vi "Main.vi"() -> ()   [LabVIEW 2026]
uses:
  <vilib>/Instr/_visa.llb/VISA Configure Serial Port (Instr).vi
panel:
  out "Errores CRC":dbl
  out "Tramas OK":dbl
  out "Estado":string
  out "SALIDA PWM":dbl(graph)
  in  "Modo":bool=TRUE
  in  "RESET":bool
  out "Maquina":T1(ring)
  in  "EMERGENCIA":bool
  in  "PWM":dbl min=0.0 max=100.0
  out "SP Vs ALTURA":cluster{dbl, dbl}(graph)
  out "PING PONG":dbl(slide) scale=0.0..50.0
  out "PID":enum16{"NO CONFIGURADO", "CONFIGURADO"}(ring)
  out "error out":errorcluster
  out "Enum":enum16{"DESCONECTADO", "CONECTADO"}(ring)
  out "ESTADO  SYS":enum16{"DETENIDO", "EJECUTANDO", "ERROR"}(ring)
  in  "PARADA":bool
  in  "INICIO":bool
  out "PID":string
  in  "SP":dbl=25.0 min=0.0 max=100.0
  in  "KD":dbl=0.07 min=0.0 max=65535.0
  in  "KI":dbl=0.14 min=0.0 max=65535.0
  in  "KP":dbl=3.9 min=0.0 max=65535.0
  in  "PID":bool
  out "PWM":dbl format="%.2g"
  out "ERROR":dbl format="%.2g"
  out "ALTURA":dbl format="%.2g"
  out "SP":dbl format="%.2f"
  out "array":string[][](array[string])
  out "Procesar":string
  in  "Stop Simulation":bool
  in  "Numeric":u32=115200
  in  "VISA resource name":refnum<visa-resource-name>="COM12"
  out "Iteracion":i32
  # "Sistema Levitador Neumático"
  # "Planta"
  # "Grafico en Tiempo Real"
  # "COMUNICACIÓN"
  # "ESTADO DEL SISTEMA"
  # "Estado :"
  # "Puerto :"
  # "Comunicación :"
  # "Baud :"
  # "Estado PID :"
  # "CONFIGURACIÓN PID"
  # "VARIABLES EN TIEMPO REAL"
  # "KP :"
  # "KI  :"
  # "KD :"
  # "AUTO"
  # "MANUAL"
  # "SP :"
  # "PWM :"
  # "Mensaje a Procesar :"
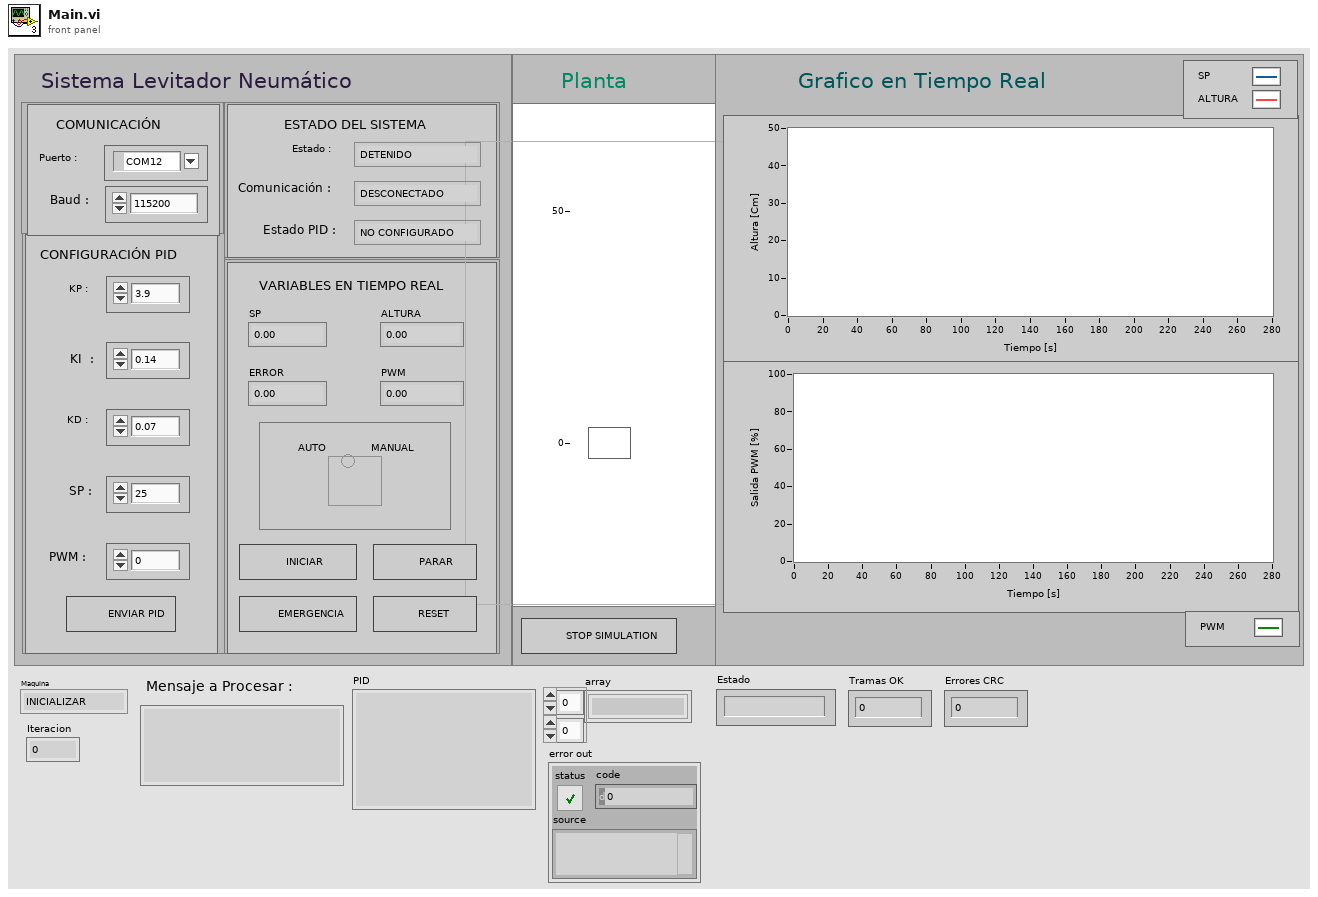
[diagram p1: front panel]
types:
  T1 = enum16{"INICIALIZAR", "ESPERA", "ENVIAR_MODO", "ENVIAR_SP", "ENVIAR_PID", "RECIBIR", "PROCESAR", "ENVIAR_RESET", "ENVIAR_RUN", "ENVIAR_STOP", "ENVIAR_EMERGENCIA_ON", "ENVIAR_EMERGENCIA_OFF", "ERROR", "CERRAR"}
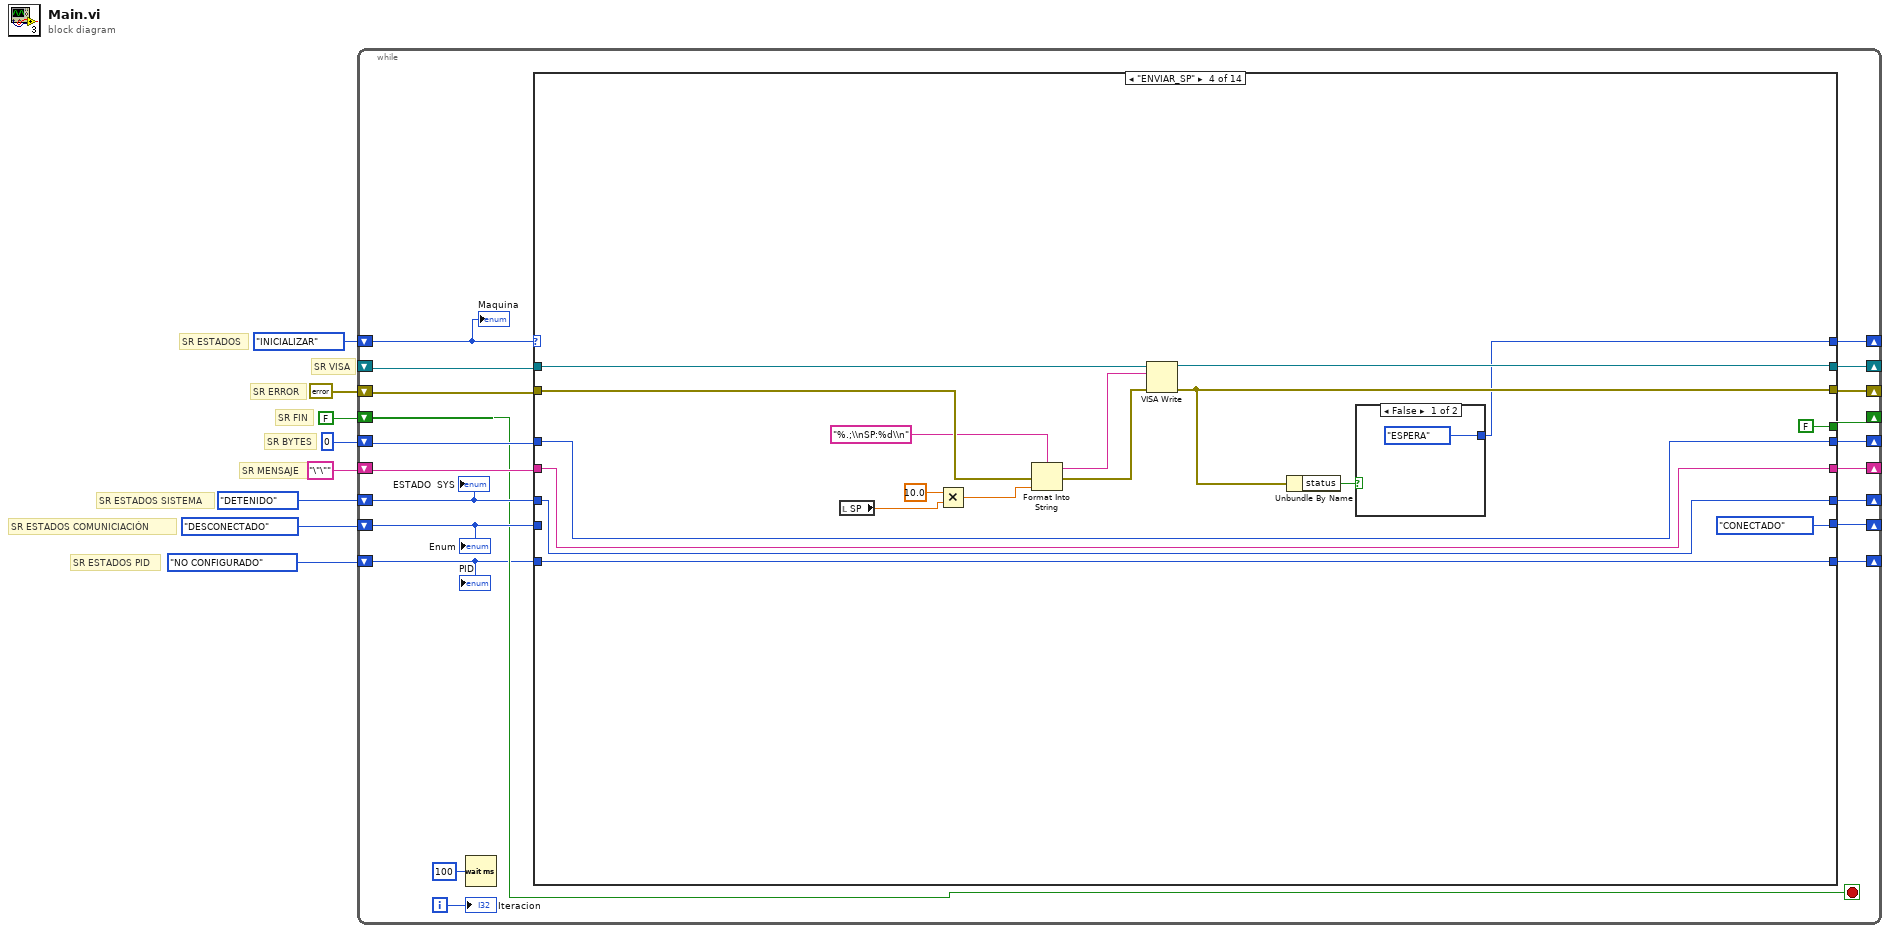
[diagram p0: block diagram]
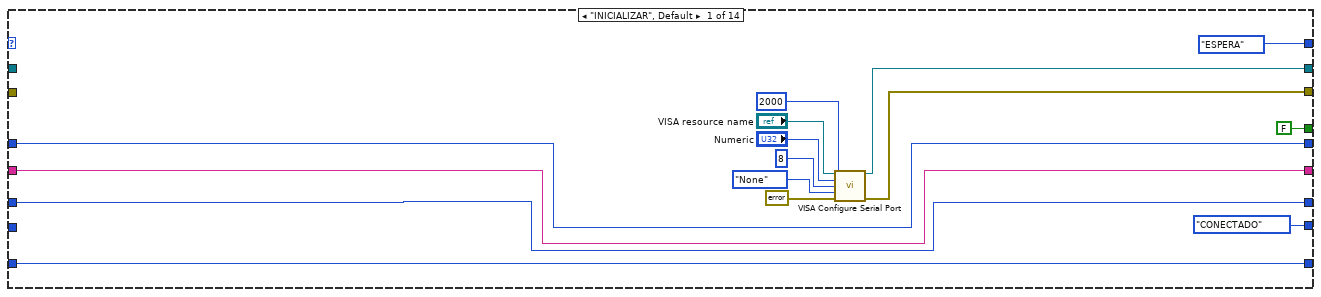
[diagram p2: hidden frame]
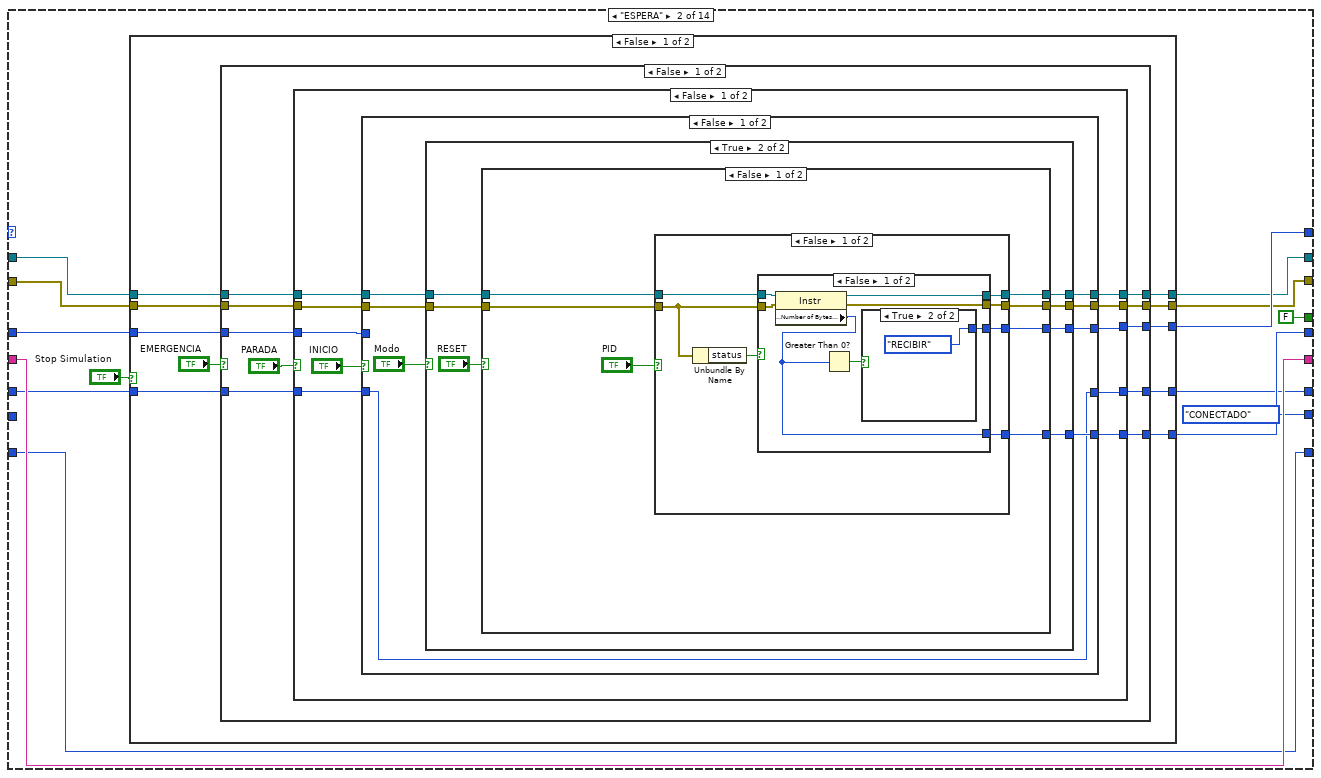
[diagram p3: hidden frame]
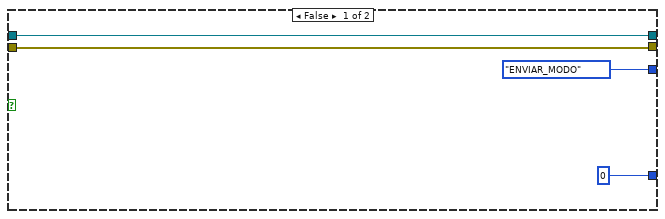
[diagram p4: hidden frame]
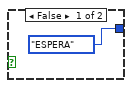
[diagram p5: hidden frame]
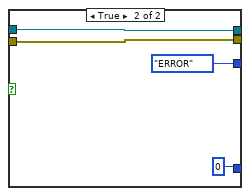
[diagram p6: hidden frame]
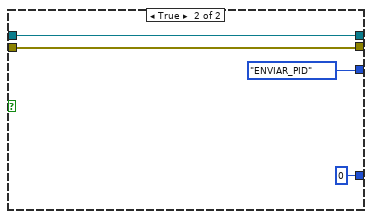
[diagram p7: hidden frame]
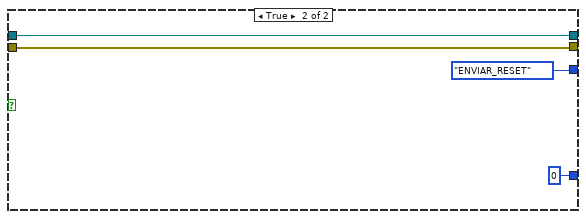
[diagram p8: hidden frame]
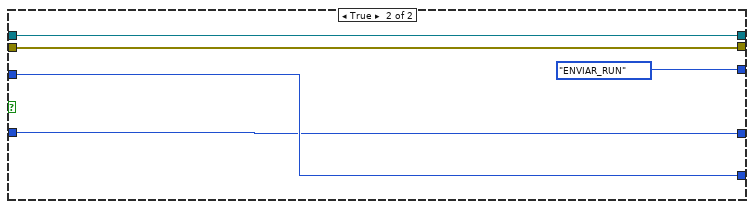
[diagram p9: hidden frame]
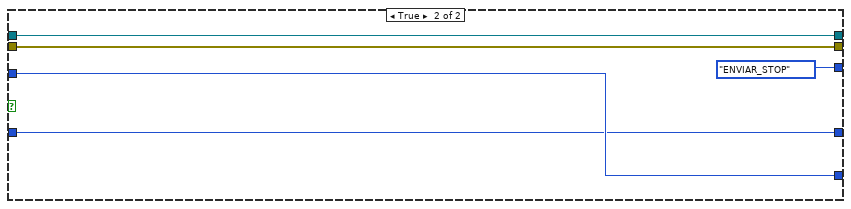
[diagram p10: hidden frame]
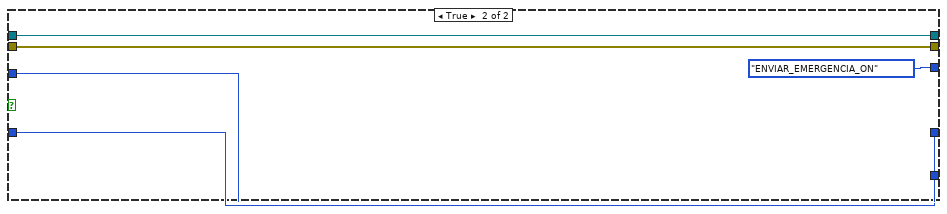
[diagram p11: hidden frame]
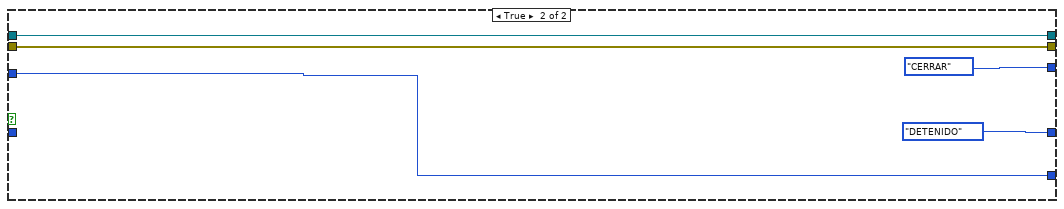
[diagram p12: hidden frame]
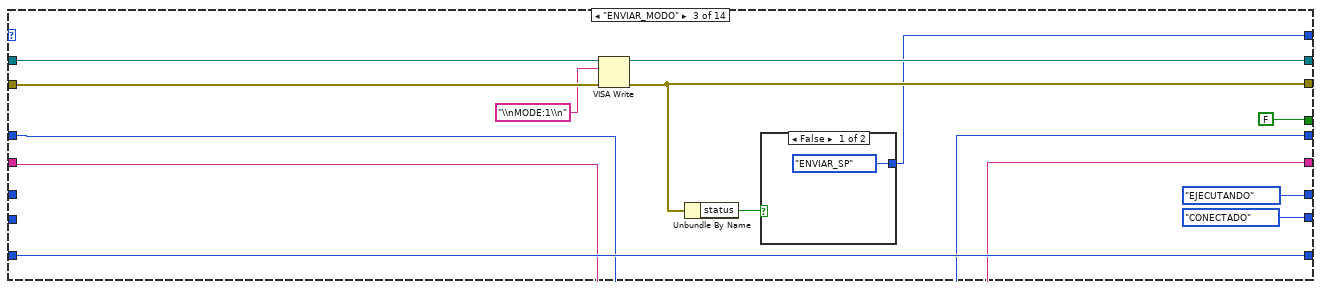
[diagram p13: hidden frame]
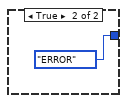
[diagram p14: hidden frame]
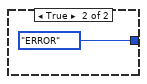
[diagram p15: hidden frame]
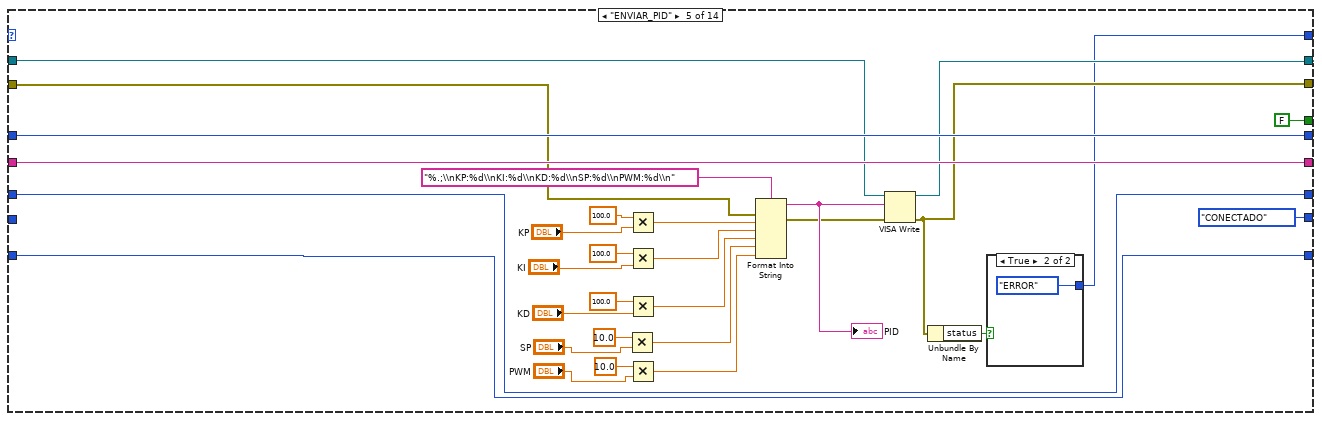
[diagram p16: hidden frame]
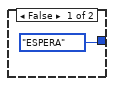
[diagram p17: hidden frame]
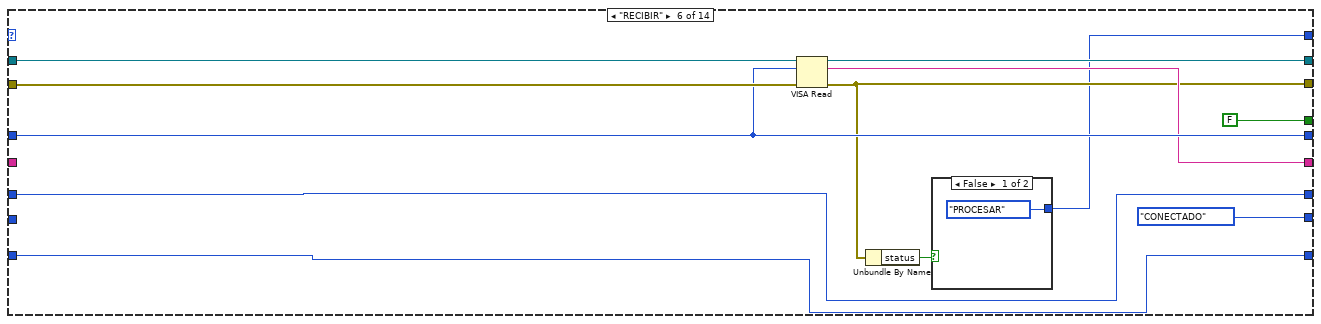
[diagram p18: hidden frame]
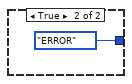
[diagram p19: hidden frame]
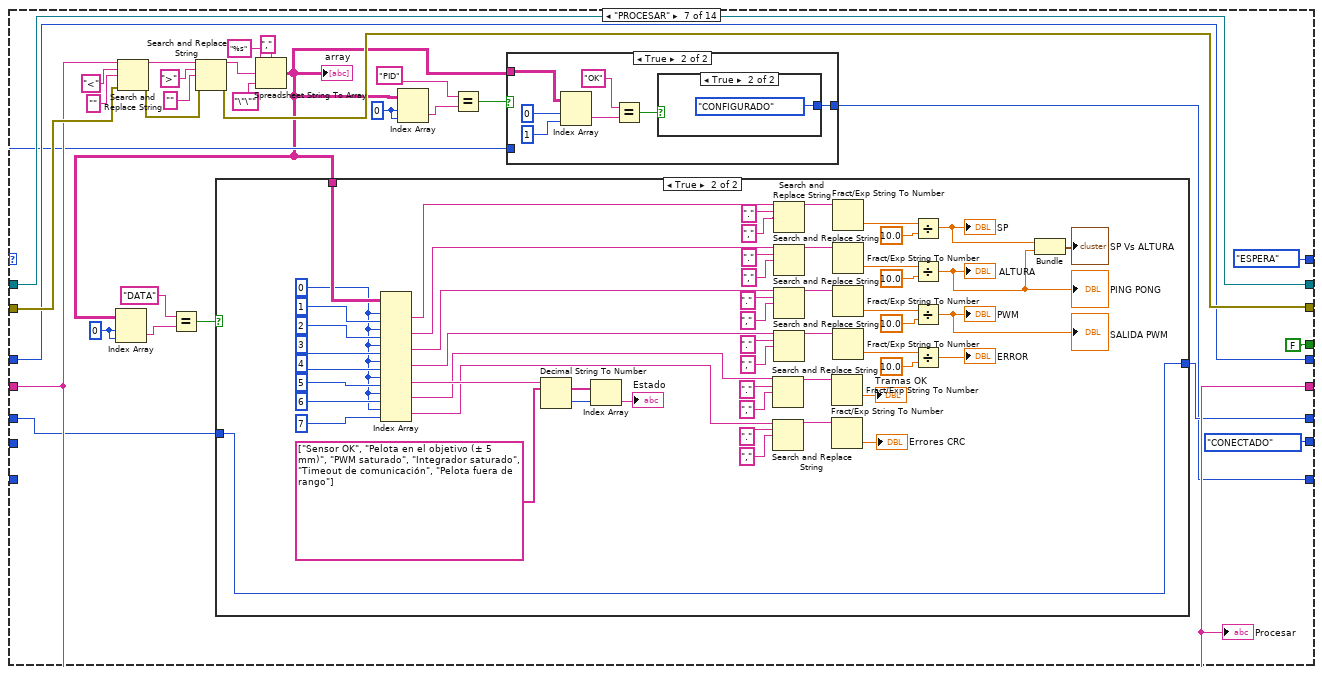
[diagram p20: hidden frame]
diagram:
  # "SR ESTADOS PID"
  # "SR ESTADOS COMUNICIACIÓN"
  # "SR ESTADOS SISTEMA"
  # "SR MENSAJE"
  # "SR BYTES"
  # "SR FIN"
  # "SR ERROR"
  # "SR ESTADOS"
  # "SR VISA"
  n1 = while {
    shift-right: [w26] -> _
    shift-left: _ -> [w24]
    shift-right: [w25] -> _
    shift-left: errorcluster {"status"=FALSE, "code"=0, "source"=""} ("error out") -> [w23]
    shift-right: [w22] -> _
    shift-left: FALSE -> [w13]
    shift-right: [w21] -> _
    shift-left: u32 0 ("Bytes at Port") -> [w20]
    shift-right: [w19] -> _
    shift-left: "\"\"" -> [w18]
    shift-right: [w14] -> _
    shift-left: enum16{"DETENIDO", "EJECUTANDO", "ERROR"}."DETENIDO" -> [w16]
    shift-right: [w15] -> _
    shift-left: enum16{"DESCONECTADO", "CONECTADO"}."DESCONECTADO" -> [w17]
    shift-right: [w11] -> _
    shift-left: enum16{"NO CONFIGURADO", "CONFIGURADO"}."NO CONFIGURADO" -> [w12]
    shift-right: [w9] -> _
    shift-left: T1."INICIALIZAR" -> [w10]
    i -> [w28]
    stop <- w13 stop-if-true
    n2 = Wait (ms)(milliseconds to wait=u32 100) -> ()  [unwired: 1 out]
    n3 = case shown="\"ENVIAR_SP\"" w10 {
      tunnel: [T1."ESPERA" w57 w167 w183 w215 w232 T1."ESPERA" w351 w370 w383 w399 w415 T1."CERRAR" T1."CERRAR"] -> w9
      tunnel: [w37 w54 w168 w192 w220 w237 w273 w354 w372 w384 w396 w417 w432 w435] -> w26
      tunnel: [w36 w53 w169 w191 w217 w234 w264 w346 w371 w385 w395 w416 w427 w436] -> w25
      tunnel: w24 -> [_ w55 w171 w194 w221 w239 w273 w356 w374 w389 w401 w419 w432 w435]
      tunnel: w23 -> [_ w49 w170 w190 w223 w238 w265 w355 w373 w388 w400 w418 w427 w437]
      tunnel: [FALSE FALSE FALSE FALSE FALSE FALSE FALSE FALSE FALSE FALSE FALSE FALSE FALSE TRUE] -> w22
      tunnel: [w34 w52 w162 w177 w225 w236 w260 w350 w367 w386 w397 w410 w430 w441] -> w21
      tunnel: w20 -> [w34 w51 w162 w177 w225 w236 w260 w350 w367 w386 w397 w410 w430 w441]
      tunnel: [w33 w50 w163 w178 w224 w235 w257 w349 w368 w387 w394 w409 w429 w440] -> w19
      tunnel: w18 -> [w33 w50 w163 w178 w224 _ w257 w349 w368 w387 w394 w409 w429 w440]
      tunnel: w16 -> [w31 w46 _ w180 w213 w230 w251 w348 _ _ _ _ w426 _]
      tunnel: w17 -> [_ _ _ _ _ _ _ _ _ _ _ _ _ _]
      tunnel: [enum16{"DESCONECTADO", "CONECTADO"}."CONECTADO" enum16{"DESCONECTADO", "CONECTADO"}."CONECTADO" enum16{"DESCONECTADO", "CONECTADO"}."CONECTADO" enum16{"DESCONECTADO", "CONECTADO"}."CONECTADO" enum16{"DESCONECTADO", "CONECTADO"}."CONECTADO" enum16{"DESCONECTADO", "CONECTADO"}."CONECTADO" enum16{"DESCONECTADO", "CONECTADO"}."CONECTADO" enum16{"DESCONECTADO", "CONECTADO"}."CONECTADO" enum16{"DESCONECTADO", "CONECTADO"}."CONECTADO" enum16{"DESCONECTADO", "CONECTADO"}."CONECTADO" enum16{"DESCONECTADO", "CONECTADO"}."CONECTADO" enum16{"DESCONECTADO", "CONECTADO"}."CONECTADO" enum16{"DESCONECTADO", "CONECTADO"}."CONECTADO" enum16{"DESCONECTADO", "CONECTADO"}."DESCONECTADO"] -> w15
      tunnel: [w31 w47 enum16{"DETENIDO", "EJECUTANDO", "ERROR"}."EJECUTANDO" w180 w213 w230 w252 w348 enum16{"DETENIDO", "EJECUTANDO", "ERROR"}."EJECUTANDO" enum16{"DETENIDO", "EJECUTANDO", "ERROR"}."DETENIDO" enum16{"DETENIDO", "EJECUTANDO", "ERROR"}."DETENIDO" enum16{"DETENIDO", "EJECUTANDO", "ERROR"}."EJECUTANDO" w426 enum16{"DETENIDO", "EJECUTANDO", "ERROR"}."DETENIDO"] -> w14
      tunnel: w12 -> [w30 w44 w164 w181 w212 w229 w245 w347 w364 w379 w398 w411 w425 w434]
      tunnel: [w30 w44 w164 w181 w212 w229 w246 w347 w364 w379 w398 w411 w425 w434] -> w11
      frame "INICIALIZAR", Default {
        n4 = call-poly "VISA Configure Serial Port"("VISA resource name"="VISA resource name", "timeout (10sec)"=u32 2000, "baud rate (9600)"="Numeric", "data bits (8)"=u16 8, "parity (0:none)"=enum16{"None", "Odd", "Even", "Mark", "Space"}."None", "error in (no error)"=errorcluster {"status"=FALSE, "code"=0, "source"=""}) -> ("VISA resource name out"=w37:refnum<visa-resource-name>, "error out"=w36:errorcluster)  [unwired: 8 in]
      }
      frame "ESPERA" {
        n5 = case shown="False" "Stop Simulation" {
          tunnel: [w67 T1."CERRAR"] -> w57
          tunnel: w55 -> [w66 w159]
          tunnel: [w65 w159] -> w54
          tunnel: [w64 w158] -> w53
          tunnel: [w63 w161] -> w52
          tunnel: w51 -> [w62 w161]
          tunnel: w49 -> [w61 w158]
          tunnel: [w60 enum16{"DETENIDO", "EJECUTANDO", "ERROR"}."DETENIDO"] -> w47
          tunnel: w46 -> [w59 _]
          frame False {
            n6 = case shown="False" "EMERGENCIA" {
              tunnel: [w77 T1."ENVIAR_EMERGENCIA_ON"] -> w67
              tunnel: w66 -> [w69 w154]
              tunnel: [w76 w154] -> w65
              tunnel: [w75 w153] -> w64
              tunnel: [w74 w156] -> w63
              tunnel: w62 -> [w73 w156]
              tunnel: w61 -> [w68 w153]
              tunnel: [w71 w155] -> w60
              tunnel: w59 -> [w70 w155]
              frame False {
                n7 = case shown="False" "PARADA" {
                  tunnel: [w87 T1."ENVIAR_STOP"] -> w77
                  tunnel: w69 -> [w86 w151]
                  tunnel: w68 -> [w85 w150]
                  tunnel: [w84 w151] -> w76
                  tunnel: [w83 w150] -> w75
                  tunnel: [w82 w149] -> w74
                  tunnel: w73 -> [w80 w149]
                  tunnel: [w79 w148] -> w71
                  tunnel: w70 -> [w78 w148]
                  frame False {
                    n8 = case shown="False" "INICIO" {
                      tunnel: [w95 T1."ENVIAR_RUN"] -> w87
                      tunnel: w86 -> [w94 w146]
                      tunnel: w85 -> [w93 w145]
                      tunnel: [w92 w146] -> w84
                      tunnel: [w91 w145] -> w83
                      tunnel: [w90 w144] -> w82
                      tunnel: w80 -> [_ w144]
                      tunnel: [w89 w143] -> w79
                      tunnel: w78 -> [w89 w143]
                      frame False {
                        n9 = case shown="True" "Modo" {
                          tunnel: [T1."ENVIAR_MODO" w106] -> w95
                          tunnel: w94 -> [w99 w105]
                          tunnel: w93 -> [w98 w104]
                          tunnel: [w99 w103] -> w92
                          tunnel: [w98 w102] -> w91
                          tunnel: [u32 0 ("Bytes at Port") w101] -> w90
                          frame False {
                          }
                          frame True {
                            n10 = case shown="False" "RESET" {
                              tunnel: [w113 T1."ENVIAR_RESET"] -> w106
                              tunnel: w105 -> [w111 w141]
                              tunnel: w104 -> [w110 w140]
                              tunnel: [w109 w141] -> w103
                              tunnel: [w108 w140] -> w102
                              tunnel: [w107 u32 0 ("Bytes at Port")] -> w101
                              frame False {
                                n11 = case shown="False" "PID" {
                                tunnel: [w120 T1."ENVIAR_PID"] -> w113
                                tunnel: w111 -> [w119 w136]
                                tunnel: w110 -> [w115 w135]
                                tunnel: [w118 w136] -> w109
                                tunnel: [w117 w135] -> w108
                                tunnel: [w116 u32 0 ("Bytes at Port")] -> w107
                                frame False {
                                n12 = Unbundle By Name(w115) -> ("status"=w114:bool)
                                n13 = case shown="False" w114 {
                                tunnel: [w127 T1."ERROR"] -> w120
                                tunnel: w119 -> [w126 w133]
                                tunnel: w115 -> [w125 w132]
                                tunnel: [w124 w133] -> w118
                                tunnel: [w123 w132] -> w117
                                tunnel: [w121 u32 0 ("Bytes at Port")] -> w116
                                frame False {
                                n14 = property class="Instr"(reference=w126, error in=w125) -> (reference out=w124:refnum<visa-resource-name>, error out=w123:errorcluster, "Serial Settings:Number of Bytes at Serial Port"=w121:u32)
                                n15 = Greater Than 0?(x=w121) -> (x > 0?=w122:bool)
                                n16 = case shown="True" w122 {
                                tunnel: [T1."ESPERA" T1."RECIBIR"] -> w127
                                frame False {
                                }
                                frame True {
                                }
                                }
                                }
                                frame True {
                                }
                                }
                                }
                                frame True {
                                }
                                }
                              }
                              frame True {
                              }
                            }
                          }
                        }
                      }
                      frame True {
                      }
                    }
                  }
                  frame True {
                  }
                }
              }
              frame True {
              }
            }
          }
          frame True {
          }
        }
      }
      frame "ENVIAR_MODO" {
        n17 = VISA Write(VISA resource name=w171, write buffer="\\nMODE:1\\n", error in (no error)=w170) -> (VISA resource name out=w168:refnum<visa-resource-name>, error out=w169:errorcluster)  [unwired: 1 out]
        n18 = Unbundle By Name(w169) -> ("status"=w165:bool)
        n19 = case shown="False" w165 {
          tunnel: [T1."ENVIAR_SP" T1."ERROR"] -> w167
          frame False {
          }
          frame True {
          }
        }
      }
      frame "ENVIAR_SP" {
        n20 = local read "SP"() -> (w186:dbl)
        n21 = Multiply(x=10.0, y=w186) -> (x*y=w188:dbl)
        n22 = Format Into String(format string="%.;\\nSP:%d\\n", error in=w190, w188) -> (resulting string=w184:string, error out=w185:errorcluster)  [unwired: 1 in]
        n23 = VISA Write(VISA resource name=w194, write buffer=w184, error in (no error)=w185) -> (VISA resource name out=w192:refnum<visa-resource-name>, error out=w191:errorcluster)  [unwired: 1 out]
        n24 = Unbundle By Name(w191) -> ("status"=w193:bool)
        n25 = case shown="False" w193 {
          tunnel: [T1."ESPERA" T1."ERROR"] -> w183
          frame False {
          }
          frame True {
          }
        }
      }
      frame "ENVIAR_PID" {
        n26 = Multiply(x=10.0, y="SP") -> (x*y=w200:dbl)
        n27 = Multiply(x=100.0, y="KP") -> (x*y=w203:dbl)
        n28 = Multiply(x=100.0, y="KI") -> (x*y=w207:dbl)
        n29 = Multiply(x=100.0, y="KD") -> (x*y=w211:dbl)
        n30 = Multiply(x=10.0, y="PWM") -> (x*y=w197:dbl)
        n31 = Format Into String(format string="%.;\\nKP:%d\\nKI:%d\\nKD:%d\\nSP:%d\\nPWM:%d\\n", error in=w223, w203, w207, w211, w200, w197) -> (resulting string=w222:string, error out=w218:errorcluster)  [unwired: 1 in]
        "PID" <- w222
        n32 = VISA Write(VISA resource name=w221, write buffer=w222, error in (no error)=w218) -> (VISA resource name out=w220:refnum<visa-resource-name>, error out=w217:errorcluster)  [unwired: 1 out]
        n33 = Unbundle By Name(w217) -> ("status"=w216:bool)
        n34 = case shown="True" w216 {
          tunnel: [T1."ESPERA" T1."ERROR"] -> w215
          frame False {
          }
          frame True {
          }
        }
      }
      frame "RECIBIR" {
        n35 = VISA Read(VISA resource name=w239, byte count=w236, error in (no error)=w238) -> (VISA resource name out=w237:refnum<visa-resource-name>, read buffer=w235:string, error out=w234:errorcluster)  [unwired: 1 out]
        n36 = Unbundle By Name(w234) -> ("status"=w233:bool)
        n37 = case shown="False" w233 {
          tunnel: [T1."PROCESAR" T1."ERROR"] -> w232
          frame False {
          }
          frame True {
          }
        }
      }
      frame "PROCESAR" {
        w250 = 0 ("index (row)")
        w256 = 0 ("index (row)")
        n38 = Search and Replace String(input string=w257, search string="<", replace string="" ("replace string (\"\")"), error in=w265) -> (result string=w269:string, error out=w268:errorcluster)  [unwired: 4 in, 2 out]
        n39 = Search and Replace String(input string=w269, search string=">", replace string="" ("replace string (\"\")"), error in=w268) -> (result string=w262:string, error out=w264:errorcluster)  [unwired: 4 in, 2 out]
        n40 = Spreadsheet String To Array(delimiter (Tab)=",", format string="%s", spreadsheet string=w262, array type (2D Dbl)="\"\"") -> (array=w243:string[][])
        "array" <- w243
        n41 = Index Array(array=w243, index (row)=w256, index (col)=w256) -> (element=w255:string)
        n42 = Equal?(x="DATA", y=w255) -> (x = y?=w253:bool)
        n43 = case shown="True" w253 {
          tunnel: w243 -> [w290 w324]
          tunnel: [w284 w323] -> w252
          tunnel: w251 -> [_ w323]
          frame False {
            n44 = Index Array(array=w290, index (row)=0, index (col)=1 ("disabled index (col)")) -> (element=w287:string)
            n45 = Equal?(x="RUN", y=w287) -> (x = y?=w285:bool)
            n46 = case shown="True" w285 {
              tunnel: [enum16{"DETENIDO", "EJECUTANDO", "ERROR"}."DETENIDO" enum16{"DETENIDO", "EJECUTANDO", "ERROR"}."EJECUTANDO"] -> w284
              frame False {
              }
              frame True {
              }
            }
          }
          frame True {
            w314 = 0 ("index (row)")
            n47 = Index Array(array=w324, index (row) #1=w314, index (col) #1=1 ("index"), index (row) #2=w314, index (col) #2=2 ("index"), index (row) #3=w314, index (col) #3=3 ("index"), index (row) #4=w314, index (col) #4=4 ("index"), index (row) #5=w314, index (col) #5=5 ("disabled index (col)"), index (row) #6=w314, index (col) #6=6 ("disabled index (col)"), index (row) #7=w314, index (col) #7=7 ("disabled index (col)")) -> (element #1=w341:string, element #2=w332:string, element #3=w331:string, element #4=w330:string, element #5=w319:string, element #6=w306:string, element #7=w305:string)
            n48 = Decimal String To Number(string=w319) -> (number=w317:i32)  [unwired: 2 in, 1 out]
            n49 = Index Array(array=string[] ["Sensor OK", "Pelota en el objetivo (± 5 mm)", "PWM saturado", "Integrador saturado", "Timeout de comunicación", "Pelota fuera de rango"], index=w317) -> (element=→"Estado":string)
            n50 = Search and Replace String(input string=w306, search string=".", replace string="," ("replace string (\"\")")) -> (result string=w308:string)  [unwired: 5 in, 3 out]
            n51 = Search and Replace String(input string=w305, search string=".", replace string="," ("replace string (\"\")")) -> (result string=w307:string)  [unwired: 5 in, 3 out]
            n52 = Search and Replace String(input string=w341, search string=".", replace string="," ("replace string (\"\")")) -> (result string=w339:string)  [unwired: 5 in, 3 out]
            n53 = Search and Replace String(input string=w332, search string=".", replace string="," ("replace string (\"\")")) -> (result string=w328:string)  [unwired: 5 in, 3 out]
            n54 = Search and Replace String(input string=w331, search string=".", replace string="," ("replace string (\"\")")) -> (result string=w327:string)  [unwired: 5 in, 3 out]
            n55 = Search and Replace String(input string=w330, search string=".", replace string="," ("replace string (\"\")")) -> (result string=w326:string)  [unwired: 5 in, 3 out]
            n56 = Fract/Exp String To Number(string=w308) -> (number=→"Tramas OK":dbl)  [unwired: 3 in, 1 out]
            n57 = Fract/Exp String To Number(string=w307) -> (number=→"Errores CRC":dbl)  [unwired: 3 in, 1 out]
            n58 = Fract/Exp String To Number(string=w339) -> (number=w321:dbl)  [unwired: 3 in, 1 out]
            n59 = Fract/Exp String To Number(string=w328) -> (number=w300:dbl)  [unwired: 3 in, 1 out]
            n60 = Fract/Exp String To Number(string=w327) -> (number=w297:dbl)  [unwired: 3 in, 1 out]
            n61 = Fract/Exp String To Number(string=w326) -> (number=w294:dbl)  [unwired: 3 in, 1 out]
            n62 = Divide(x=w321, y=10.0) -> (x/y=w302:dbl)
            "SP" <- w302
            n63 = Divide(x=w300, y=10.0) -> (x/y=w299:dbl)
            "ALTURA" <- w299
            "PING PONG" <- w299
            n64 = Divide(x=w297, y=10.0) -> (x/y=→"PWM" →"SALIDA PWM":dbl)
            n65 = Divide(x=w294, y=10.0) -> (x/y=→"ERROR":dbl)
            n66 = Bundle(w302, w299) -> (→"SP Vs ALTURA":cluster{dbl, dbl})  [unwired: 1 in]
          }
        }
        n67 = Index Array(array=w243, index (row)=w250, index (col)=w250) -> (element=w249:string)
        n68 = Equal?(x="PID", y=w249) -> (x = y?=w247:bool)
        n69 = case shown="True" w247 {
          tunnel: w243 -> [_ w277]
          tunnel: [w274 w275] -> w246
          tunnel: w245 -> [w274 _]
          frame False {
          }
          frame True {
            n70 = Index Array(array=w277, index (row)=0, index (col)=1 ("disabled index (col)")) -> (element=w279:string)
            n71 = Equal?(x="OK", y=w279) -> (x = y?=w276:bool)
            n72 = case shown="True" w276 {
              tunnel: [enum16{"NO CONFIGURADO", "CONFIGURADO"}."NO CONFIGURADO" enum16{"NO CONFIGURADO", "CONFIGURADO"}."CONFIGURADO"] -> w275
              frame False {
              }
              frame True {
              }
            }
          }
        }
        "Procesar" <- w257
      }
      frame "ENVIAR_RESET" {
        w357 = 0.0 ("input 1")
        n73 = Format Into String(format string="%.;\\nKP:%d\\nKI:%d\\nKD:%d\\nSP:%d\\nPWM:%d\\n", error in=w355, w357, w357, w357, w357, w357) -> (resulting string=w361:string, error out=w359:errorcluster)  [unwired: 1 in]
        n74 = VISA Write(VISA resource name=w356, write buffer=w361, error in (no error)=w359) -> (VISA resource name out=w354:refnum<visa-resource-name>, error out=w346:errorcluster)  [unwired: 1 out]
        n75 = Unbundle By Name(w346) -> ("status"=w358:bool)
        n76 = case shown="False" w358 {
          tunnel: [T1."ESPERA" T1."ERROR"] -> w351
          frame False {
          }
          frame True {
          }
        }
      }
      frame "ENVIAR_RUN" {
        n77 = VISA Write(VISA resource name=w374, write buffer="\\nEN:1\\n", error in (no error)=w373) -> (VISA resource name out=w372:refnum<visa-resource-name>, error out=w371:errorcluster)  [unwired: 1 out]
        n78 = Unbundle By Name(w371) -> ("status"=w376:bool)
        n79 = case shown="True" w376 {
          tunnel: [T1."ESPERA" T1."ERROR"] -> w370
          frame False {
          }
          frame True {
          }
        }
      }
      frame "ENVIAR_STOP" {
        n80 = VISA Write(VISA resource name=w389, write buffer="\\nEN:0\\n", error in (no error)=w388) -> (VISA resource name out=w384:refnum<visa-resource-name>, error out=w385:errorcluster)  [unwired: 1 out]
        n81 = Unbundle By Name(w385) -> ("status"=w391:bool)
        n82 = case shown="True" w391 {
          tunnel: [T1."ESPERA" T1."ERROR"] -> w383
          frame False {
          }
          frame True {
          }
        }
      }
      frame "ENVIAR_EMERGENCIA_ON" {
        n83 = VISA Write(VISA resource name=w401, write buffer="\\nEMG:1\\n", error in (no error)=w400) -> (VISA resource name out=w396:refnum<visa-resource-name>, error out=w395:errorcluster)  [unwired: 1 out]
        n84 = Unbundle By Name(w395) -> ("status"=w406:bool)
        n85 = case shown="False" w406 {
          tunnel: [T1."ESPERA" T1."ERROR"] -> w399
          frame False {
          }
          frame True {
          }
        }
      }
      frame "ENVIAR_EMERGENCIA_OFF" {
        n86 = VISA Write(VISA resource name=w419, write buffer="\\nEMG:0\\n", error in (no error)=w418) -> (VISA resource name out=w417:refnum<visa-resource-name>, error out=w416:errorcluster)  [unwired: 1 out]
        n87 = Unbundle By Name(w416) -> ("status"=w421:bool)
        n88 = case shown="False" w421 {
          tunnel: [T1."ESPERA" T1."ERROR"] -> w415
          frame False {
          }
          frame True {
          }
        }
      }
      frame "ERROR" {
        "error out" <- w427
      }
      frame "CERRAR" {
        n89 = VISA Close(VISA resource name=w435, error in (no error)=w437) -> (error out=w436:errorcluster)
      }
    }
    "Iteracion" <- w28
    "ESTADO  SYS" <- w16
    "Enum" <- w17
    "PID" <- w12
    "Maquina" <- w10
  }
